vi "Port Address.vi"(8 "error in":errorcluster) -> (0 "error out":errorcluster, 2 "Visa Resource":refnum<visa-resource-name>, 3 "text":string)   [LabVIEW 2026]
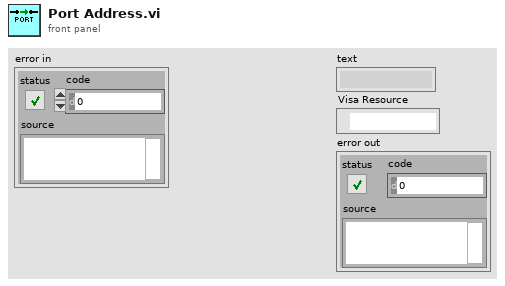
[diagram p1: front panel]
types:
  T1 = enum16{"open", "replace", "create", "open or create", "replace or create", "replace or create with confirmation"}
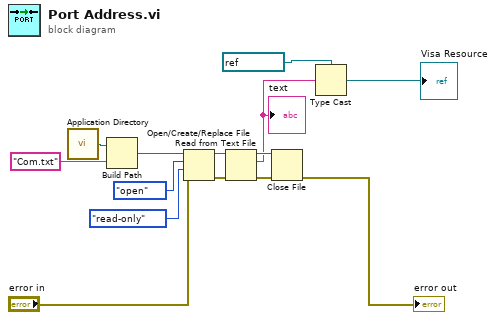
[diagram p0: block diagram]
diagram:
  n1 = call <vilib>:"Application Directory.vi"() -> ("Application Directory"=w6:path)
  n2 = Build Path(base path=w6, name or relative path="Com.txt") -> (appended path=w5:path)
  n3 = Open/Create/Replace File(file path (use dialog)=w5, error in="error in", operation (0:open)=T1."open", access (0:read/write)=enum16{"read/write", "read-only", "write-only"}."read-only") -> (refnum out=w14:refnum<file>, error out=w12:errorcluster)  [unwired: 2 in, 1 out]
  n4 = Read from Text File(file (use dialog)=w14, error in=w12) -> (refnum out=w13:refnum<file>, text=w4:string, error out=w11:errorcluster)  [unwired: 2 in, 1 out]
  "text" <- w4
  n5 = Close File(refnum=w13, error in=w11) -> (error out=→"error out":errorcluster)  [unwired: 1 out]
  n6 = Type Cast(type=refnum<visa-resource-name> "COM3" ("Com Port"), x=w4) -> (*(type *) &x=→"Visa Resource":refnum<visa-resource-name>)
